vi "Get All Test Results.vi"(6 "Filter Orphaned Tests? (F)":bool, 8 "error in (no error)":errorcluster, 11 "Test Result in":refnum<class "Test Result.lvclass">) -> (0 "error out":errorcluster, 2 "Test Results":T1[](array[typedef]), 3 "Test Result out":refnum<class "Test Result.lvclass">)   [LabVIEW 2020, in "Caraya.lvlib" / "Test Result.lvclass"]
doc: "Use the new method for any future development.\n\nReplace with \"Get All Test Results (Extended).vi\""
uses:
  Test Result.lvclass
  Node Results.ctl
  Test Node.ctl
  Test Registration Data.ctl
  Assert Event Data.ctl
  Test Result.lvclass/Test Result.ctl
  Node Results (Extended).ctl
  Test Node (Extended).ctl
  Assert Event Data (Extended).ctl
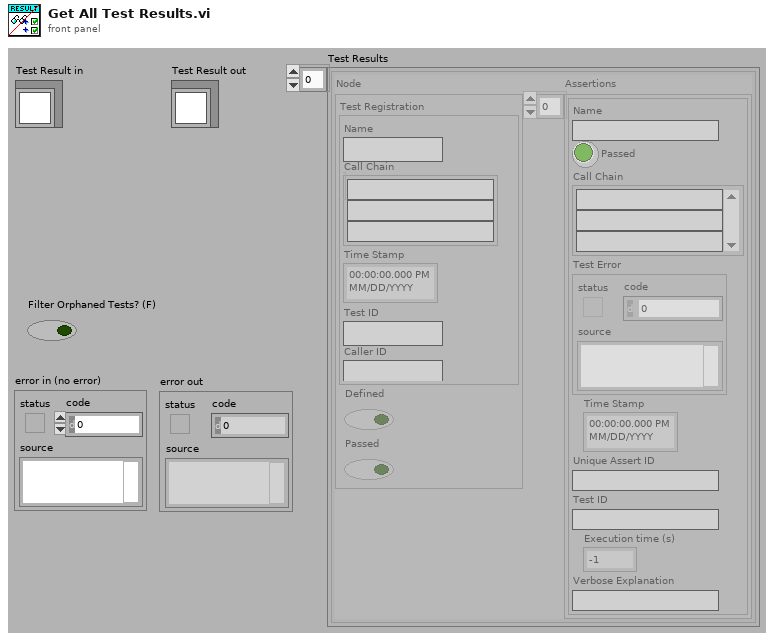
[diagram p1: front panel]
types:
  T1 = typedef "Caraya.lvlib/Test Result.lvclass/Node Results.ctl" = cluster{"Node":T2, "Assertions":T4[]}
  T2 = typedef "Caraya.lvlib/Test Result.lvclass/Test Node.ctl" = cluster{"Test Registration":T3, "Defined":bool, "Passed":bool}
  T3 = typedef "Caraya.lvlib/Test Result.lvclass/Test Registration Data.ctl" = cluster{"Name":string, "Call Chain":string[], "Time Stamp":timestamp, "Test ID":string, "Caller ID":string}
  T4 = typedef "Caraya.lvlib/Test Result.lvclass/Assert Event Data.ctl" = cluster{"Name":string, "Passed":bool, "Call Chain":string[], "Test Error":errorcluster, "Time Stamp":timestamp, "Unique Assert ID":string, "Test ID":string, "Execution time (s)":dbl, "Verbose Explanation":string}
  T5 = typedef "Caraya.lvlib/Test Result.lvclass/Node Results (Extended).ctl" = cluster{"Test Node":T6, "Assertions":T7[]}
  T6 = typedef "Caraya.lvlib/Test Result.lvclass/Test Node (Extended).ctl" = cluster{"Test Registration":T3, "Defined":bool, "Passed":bool, "properties":variant}
  T7 = typedef "Caraya.lvlib/Test Result.lvclass/Assert Event Data (Extended).ctl" = cluster{"name":string, "passed":bool, "call-chain":string[], "test-error":errorcluster, "timestamp":timestamp, "assert-id":string, "test-id":string, "time":dbl, "message":string, "properties":variant, "measurements":variant, "user-defined":variant}
  T8 = cluster{i32, "Time Stamp":timestamp, "Caller ID":string, "Test ID":string, "Node Result":T1}
  T9 = cluster{i32, "Time Stamp":timestamp, "Caller ID":string, "Test ID":string, "Node Result":T1}[]
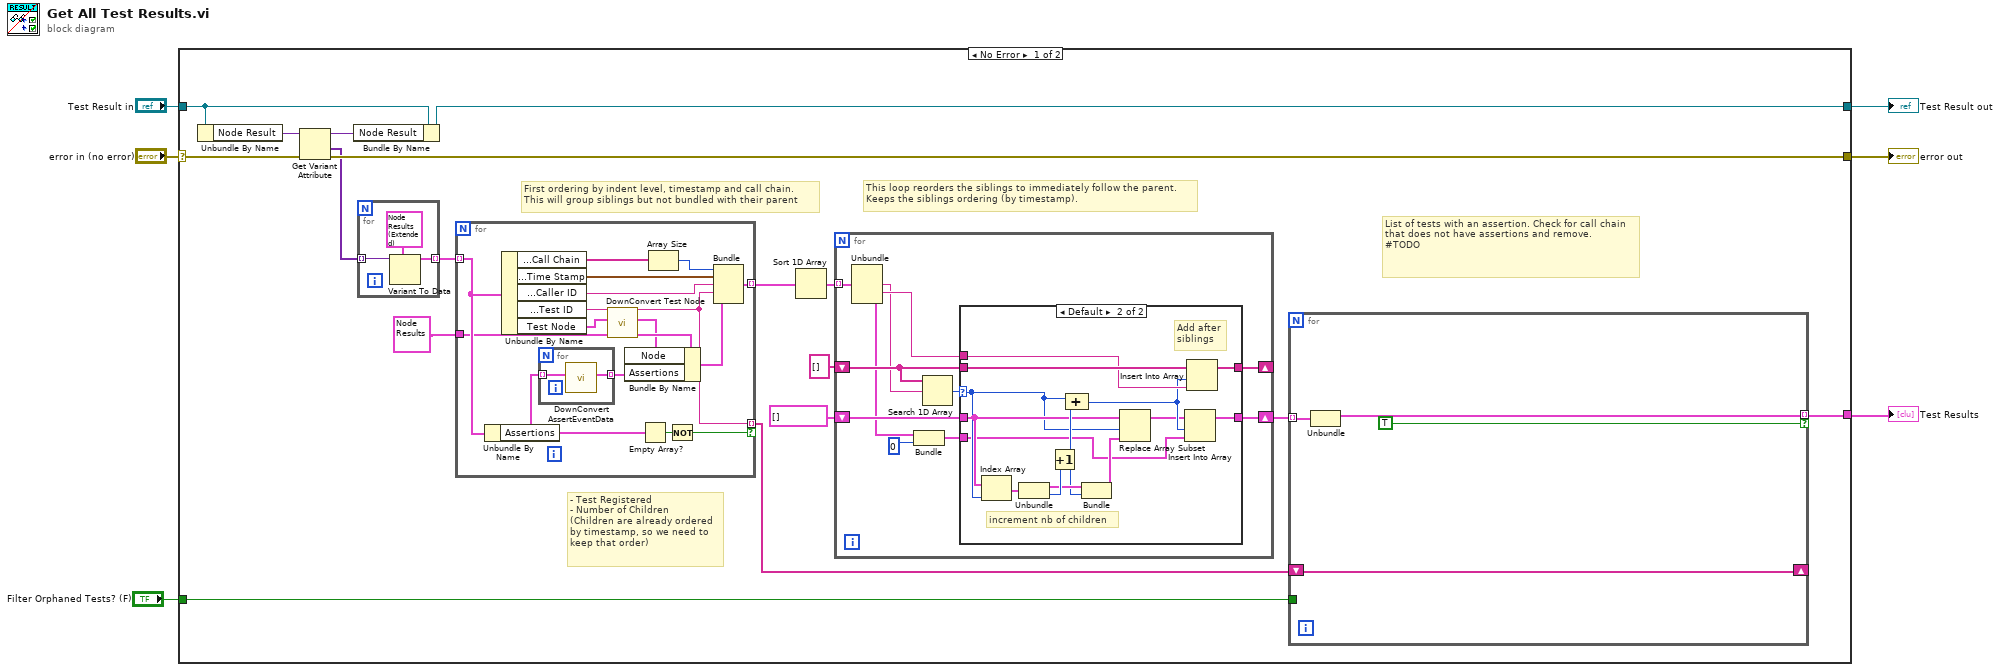
[diagram p0: block diagram]
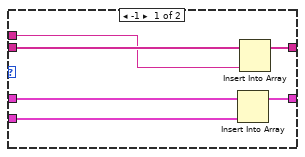
[diagram p2: hidden frame]
diagram:
  n1 = case shown="No Error" "error in (no error)" {
    selector: "error in (no error)" -> [w18 w80]
    tunnel: [w19 w80] -> w5
    tunnel: [w22 w79] -> w3
    tunnel: "Test Result in" -> [w23 w79]
    tunnel: [w10 _] -> w2
    tunnel: "Filter Orphaned Tests? (F)" -> [w8 _]
    frame No Error {
      # "List of tests with an assertion. Check for call chain that does not have assertions and remove.\n#TODO"
      # "First ordering by indent level, timestamp and call chain.\nThis will group siblings but not bundled with their parent"
      # "- Test Registered\n- Number of Children\n(Children are already ordered\nby timestamp, so we need to \nkeep that order)"
      # "This loop reorders the siblings to immediately follow the parent.\nKeeps the siblings ordering (by timestamp)."
      n2 = Unbundle By Name(w23) -> ("Node Result"=w21:variant)
      n3 = Get Variant Attribute(Variant=w21, error in=w18) -> (duplicate Variant=w20:variant, values=w17:variant[], error out=w19:errorcluster)  [unwired: 2 in, 1 out]
      n4 = Bundle By Name(cluster=w23, "Node Result"=w20) -> (w22:refnum<class "Test Result.lvclass">)
      n5 = for {
        tunnel: w17 -> [w78] mode=indexing
        tunnel: [w77] -> w16 mode=indexing
        n6 = Variant To Data(type=T5 {"Test Node"={"Test Registration"={"Name"="", "Call Chain"=[], "Time Stamp"=timestamp(0 s since 1904-01-01), "Test ID"="", "Caller ID"=""}, "Defined"=FALSE, "Passed"=FALSE, "properties"=variant}, "Assertions"=[]} ("Extended Node Result"), Variant=w78) -> (data=w77:T5)  [unwired: 1 in, 1 out]
      }
      n7 = for {
        tunnel: w16 -> [w63] mode=indexing
        tunnel: [w73] -> w14 mode=indexing
        tunnel: [w66] -> w9 mode=indexing if=w68
        tunnel: T1 {"Node"={"Test Registration"={"Name"="", "Call Chain"=[], "Time Stamp"=timestamp(0 s since 1904-01-01), "Test ID"="", "Caller ID"=""}, "Defined"=FALSE, "Passed"=FALSE}, "Assertions"=[]} ("Node Result") -> [w61]
        n8 = Unbundle By Name(w63) -> ("Assertions"=w65:T7[])
        n9 = Unbundle By Name(w63) -> ("Test Node.Test Registration.Call Chain"=w71:string[], "Test Node.Test Registration.Time Stamp"=w70:timestamp, "Test Node.Test Registration.Caller ID"=w67:string, "Test Node.Test Registration.Test ID"=w66:string, "Test Node"=w60:T6)
        n10 = for {
          tunnel: w65 -> [w75] mode=indexing
          tunnel: [w74] -> w64 mode=indexing
          n11 = call "DownConvert AssertEventData.vi"("Assert Event Data (Extended)"=w75) -> ("Assert Event Data"=w74:T4)  [unwired: 10 in]
        }
        n12 = call "DownConvert Test Node.vi"("Test Node (Extended)"=w60) -> ("Test Node"=w59:T2)  [unwired: 10 in]
        n13 = Bundle By Name(cluster=w61, "Node"=w59, "Assertions"=w64) -> (w62:T1)
        n14 = Empty Array?(array=w65) -> (empty?=w69:bool)
        n15 = Array Size(array=w71) -> (size(s)=w72:i32)
        n16 = Not(x=w69) -> (.not. x?=w68:bool)
        n17 = Bundle(w72, "Time Stamp"=w70, "Caller ID"=w67, "Test ID"=w66, "Node Result"=w62) -> (w73:T8)  [unwired: 1 in]
      }
      n18 = Sort 1D Array(array=w14) -> (sorted array=w15:T9)
      n19 = for {
        tunnel: w15 -> [w38] mode=indexing
        shift-right: [w36] -> w11
        shift-left: cluster{"Node Result":T1, i32}[] [] -> [w37]
        shift-right: [w34] -> _
        shift-left: string[] [] -> [w33]
        n20 = Unbundle(w38) -> ("Caller ID"=w29:string, "Test ID"=w30:string, "Node Result"=w28:T1)  [unwired: 2 out]
        n21 = Bundle("Node Result"=w28, 0) -> (w31:cluster{"Node Result":T1, i32})  [unwired: 1 in]
        n22 = Search 1D Array(1D array=w33, element=w29) -> (index of element=w35:i32)  [unwired: 1 in]
        n23 = case shown="Default" w35 {
          selector: w35 -> [_ w47]
          tunnel: w37 -> [w44 w49]
          tunnel: [w43 w58] -> w36
          tunnel: w31 -> [w42 w45]
          tunnel: w33 -> [w41 w57]
          tunnel: [w40 w56] -> w34
          tunnel: w30 -> [w39 w55]
          frame -1 {
            n24 = Insert Into Array(array=w44, new element=w42) -> (w43:cluster{"Node Result":T1, i32}[])  [unwired: 1 in]
            n25 = Insert Into Array(array=w41, new element=w39) -> (w40:string[])  [unwired: 1 in]
          }
          frame Default {
            # "Add after\nsiblings"
            # "increment nb of children"
            n26 = Index Array(array=w49, index=w47) -> (element=w54:cluster{"Node Result":T1, i32})
            n27 = Unbundle(w54) -> ("Node Result"=w51:T1, w53:i32)
            n28 = Increment(x=w53) -> (x+1=w50:i32)
            n29 = Compound Arithmetic op=ADD(w47, w50) -> (w52:i32)
            n30 = Bundle("Node Result"=w51, w50) -> (w46:cluster{"Node Result":T1, i32})  [unwired: 1 in]
            n31 = Replace Array Subset(array=w49, new element=w46, index=w47) -> (w48:cluster{"Node Result":T1, i32}[])
            n32 = Insert Into Array(array=w48, index=w52, new element=w45) -> (w58:cluster{"Node Result":T1, i32}[])
            n33 = Insert Into Array(array=w57, index=w52, new element=w55) -> (w56:string[])
          }
        }
      }
      n34 = for {
        tunnel: w11 -> [w27] mode=indexing
        tunnel: [w26] -> w10 mode=indexing if=TRUE
        tunnel: w8 -> [_]
        shift-right: [w24] -> _
        shift-left: w9 -> [w24]
        n35 = Unbundle(w27) -> ("Node Result"=w26:T1)  [unwired: 1 out]
      }
    }
    frame Error {
    }
  }
  "error out" <- w5
  "Test Result out" <- w3
  "Test Results" <- w2
